vi "Prog.vi"(6 "error in (no error) 2":errorcluster, 9 "base path":path) -> (0 "error out":errorcluster, 2 "Result":string, 3 "RESULT":bool)   [LabVIEW 2021]
panel:
  out "standard error":string
  out "concatenated string 2":string
  out "standard output 2":string
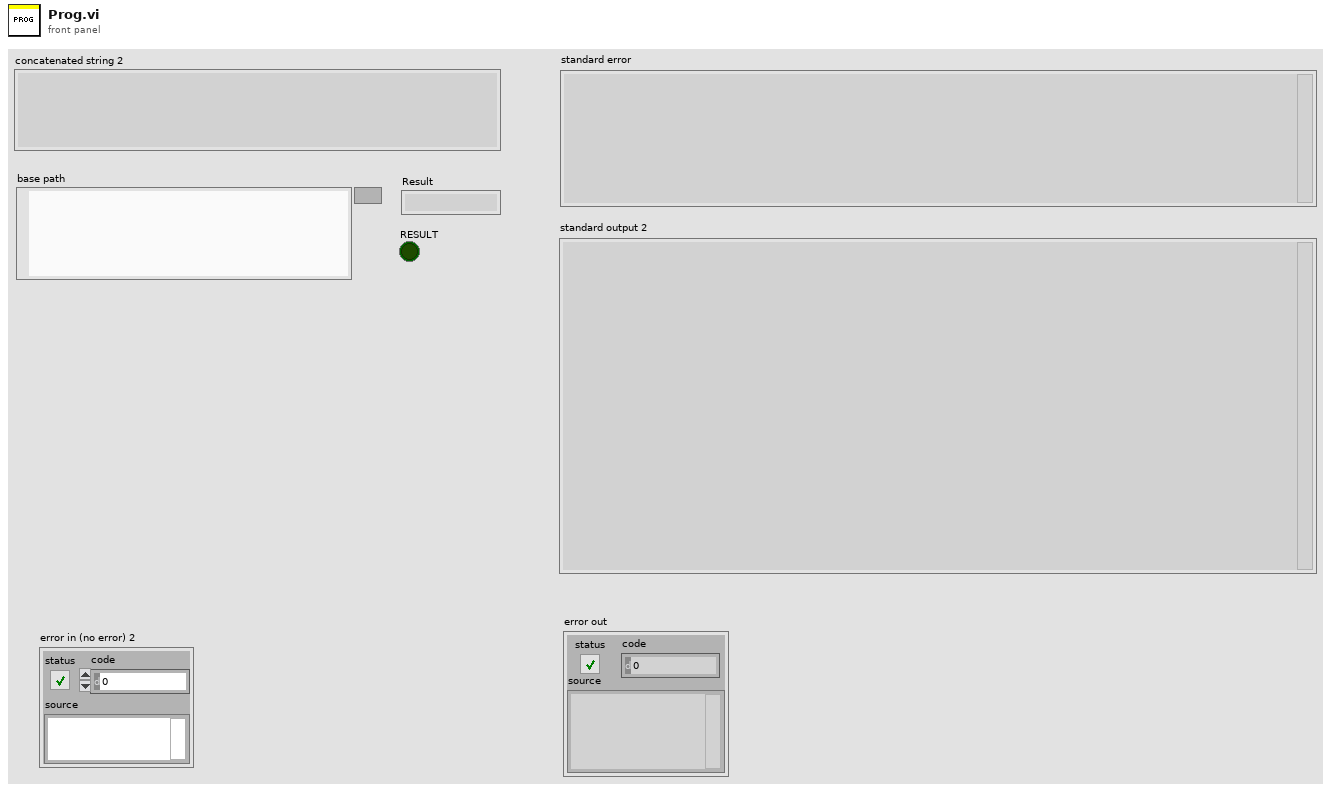
[diagram p1: front panel]
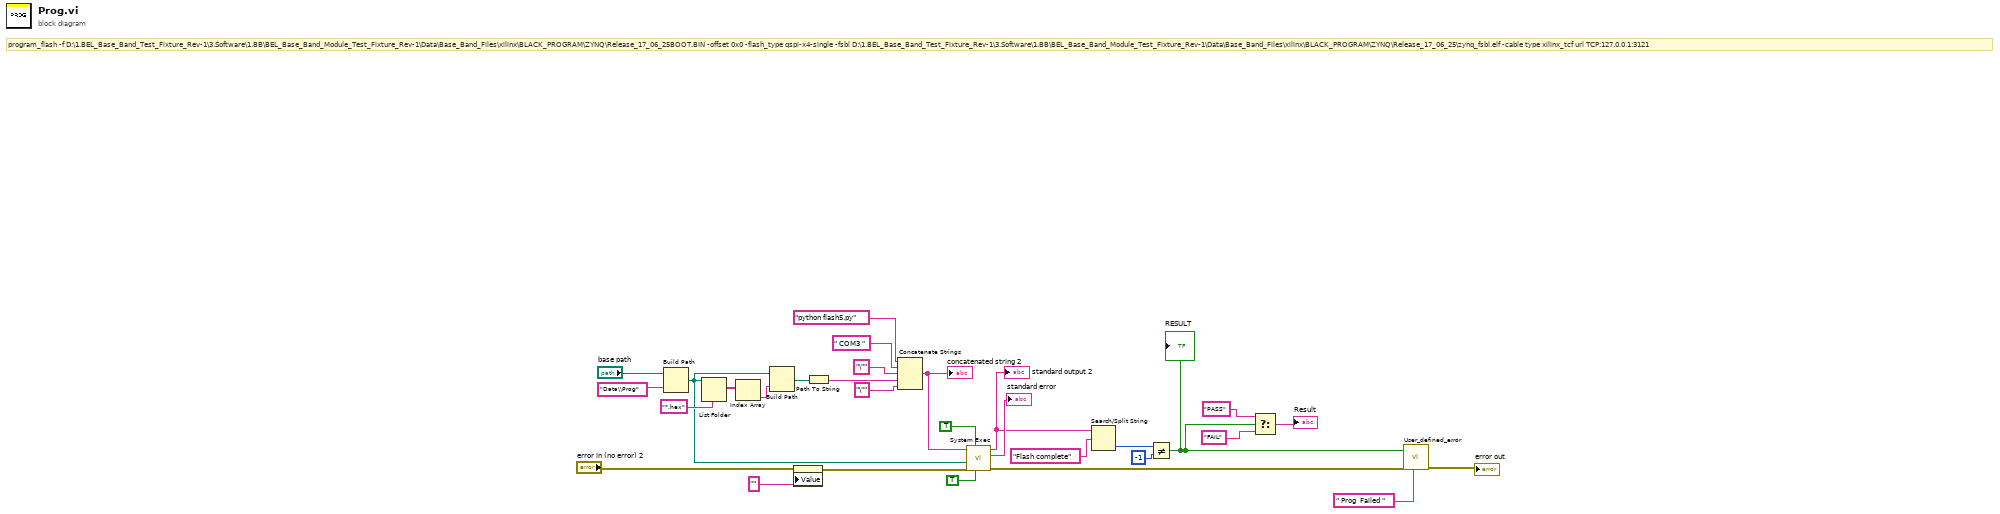
[diagram p0: block diagram]
diagram:
  # "program_flash -f D:\\1.BEL_Base_Band_Test_Fixture_Rev-1\\3.Software\\1.BB\\BEL_Base_Band_Module_Test_Fixture_Rev-1\\Data\\Base_Band_Files\\xilinx\\BLACK_PROGRAM\\ZYNQ\\Release_17_06_25BOOT.BIN -offset 0x0 -flash_type qspi-x4-single -fsbl D:\\1.BEL_Base_Band_Test_Fixture_Rev-1\\3.Software\\1.BB\\BEL_Base_Band_Module_Test_Fixture_Rev-1\\Data\\Base_Band_Files\\xilinx\\BLACK_PROGRAM\\ZYNQ\\Release_17_06_25\\zynq_fsbl.elf -cable type xilinx_tcf url TCP:127.0.0.1:3121"
  n1 = Build Path(base path="base path", name or relative path="Data\\Prog") -> (appended path=w16:path)
  n2 = List Folder(path=w16, pattern="*.hex") -> (filenames=w27:string[])  [unwired: 2 in, 3 out]
  n3 = Index Array(array=w27) -> (element=w25:string)  [unwired: 1 in]
  n4 = Build Path(base path=w16, name or relative path=w25) -> (appended path=w26:path)
  n5 = property on="standard output 2" class="Str"(error in="error in (no error) 2", "Value"="") -> (error out=w20:errorcluster)  [unwired: 1 in, 1 out]
  n6 = Path To String(path=w26) -> (string=w23:string)
  n7 = Concatenate Strings("python flash5.py", " COM3 " ("string"), "\"" ("string"), w23, "\"" ("string")) -> (w14:string)
  "concatenated string 2" <- w14
  n8 = call <vilib>:"System Exec.vi"("run minimized? (F)"=TRUE, "wait until completion? (T)"=TRUE, "error in (no error)"=w20, "working directory"=w16, "command line"=w14) -> ("error out"=w7:errorcluster, "standard error"=→"standard error":string, "standard output"=w2:string)  [unwired: 3 in, 1 out]
  "standard output 2" <- w2
  n9 = Search/Split String(string=w2, search string/char (-)="Flash complete") -> (offset of match=w12:i32)  [unwired: 1 in, 2 out]
  n10 = Not Equal?(x=w12, y=-1) -> (x != y?=w6:bool)
  "RESULT" <- w6
  n11 = Select(t="PASS", s=w6, f="FAIL") -> (s? t:f=→"Result":string)
  n12 = call "User_defined_error.vi"("Error Msg"=" Prog  Failed " ("source"), "error in"=w7, "Result"=w6) -> ("error Out"=→"error out":errorcluster)  [unwired: 8 in]
